vi "CSM-Logger-Thread.vi"(4 "Log Limit":T1={"file size (in bytes)"=10000000, "file num"=2} {"file size (in bytes)" format="%.0p"}, 6 "Exit When All Module Exist? (F)":bool, 7 "Format String":string="%<%Y/%m/%d %H:%M:%S%3u>T", 8 "error in (no error)":errorcluster, 9 "WatchDogQ":refnum<queue>, 10 "GlobalLogFilter.lvclass":refnum<class "LogFilter.lvclass">, 11 "File Path (Use Dialog)":path) -> (0 "error out":errorcluster)   [LabVIEW 2017, in "CSM File Logger.lvlib"]
doc: "The thread VI used in the CSM - Start File Logger VI.\n\n\n> [!NOTE] <b>CSM File Logger Implementation Principle</b>\n>\n> The CSM File Logger retrieves all execution records in the application via the CSM Global Log API and saves them to a specified text file for later analysis and error localization. The file format is a text file with the suffix `.csmlog`, which can be opened using text editing query tools such as Notepad."
uses:
  CSM File Logger.lvlib
  CSM File Logger Limit.ctl
  _Support/GlobalEvent/LogFilter/LogFilter.lvclass
  _Support/Typedef/_CSM_List Module Scope.ctl
  Communicable State Machine.lvlib
  _Shared/CSM Shared.lvlib
panel:
  in  "internal Stop":bool
  out "#MsgInQueue":i32
  out "size (in bytes)":i64
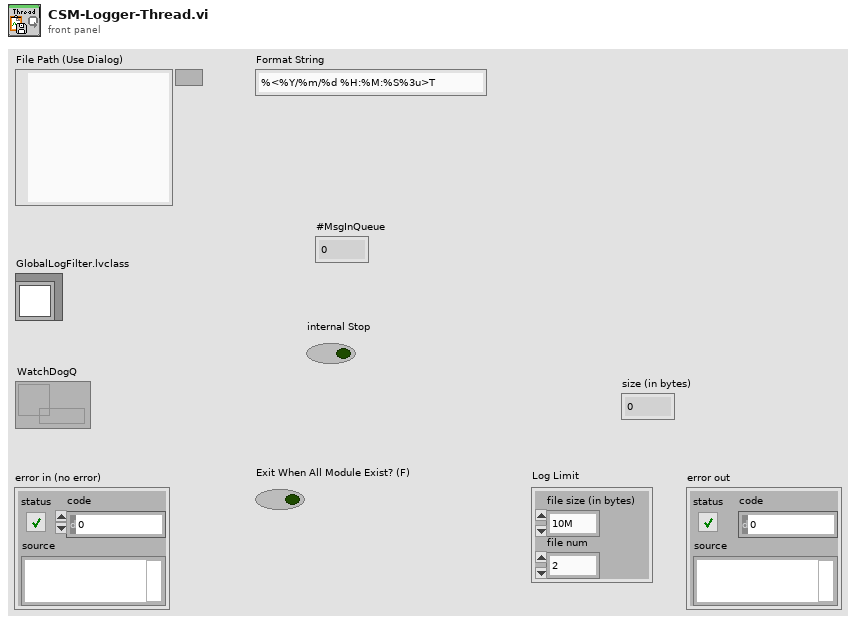
[diagram p1: front panel]
types:
  T1 = typedef "CSM File Logger.lvlib/CSM File Logger Limit.ctl" = cluster{"file size (in bytes)":i64, "file num":i32}
  T2 = typedef "Communicable State Machine.lvlib/_CSM_GlobalLog_MSG_TYPE.ctl" = enum16{"User Log", "State Change", "Status", "Interrupt", "Register", "Unregister", "Error Log", "Module Created", "Module Destroyed", "Async Message", "No-Rep Async Message", "Sync Message"}
  T3 = typedef "Communicable State Machine.lvlib/_CSM_GlobalLog_STATE_TYPE.ctl" = enum16{"State - Internal State", "State - External Message", "State - Response", "State - Complete"}
  T4 = cluster{"Global":cluster{"CSM":string[], "LogType":T2[], "State":string[], "StateType":T3[]}, "CSM":cluster{"LogType":cluster{"CSM":string, "LogType":T2}[], "State":cluster{"CSM":string, "State":string}[], "StateType":cluster{"CSM":string, "LogType":T3}[]}, "PeriodicLog":cluster{"Enable":bool, "Threshold(#/s)":dbl, "CheckPeriod(s)":dbl}}
  T5 = cluster{"Queue":path[], "folder":path, "name":string, "index":i32, "Log Limit":T1}
  T6 = enum16{"open", "replace", "create", "open or create", "replace or create", "replace or create with confirmation"}
  T7 = typedef "Communicable State Machine.lvlib/_CSM_List Module Scope.ctl" = enum16{"Normal", "System Only", "All"}
  T8 = typedef "Communicable State Machine.lvlib/Periodic String Filter Level.ctl" = enum16{"normal", "L1", "L2", "L3", "L4"}
  T9 = typedef "Communicable State Machine.lvlib/_CSM_GlobalLog_MSG.ctl" = cluster{"Name (\"\" to Use UUID)":string, "Current State":string, "Arguments":string, "Source Message":T10, "Source Module":string, "Complete(T)/Start(F)":bool, "LogType":T2, "Time Stamp":timestamp}
  T10 = typedef "Communicable State Machine.lvlib/_CSM_Response Source Message.ctl" = cluster{"‘State":string, "’Arguments":string, "’Error":errorcluster}
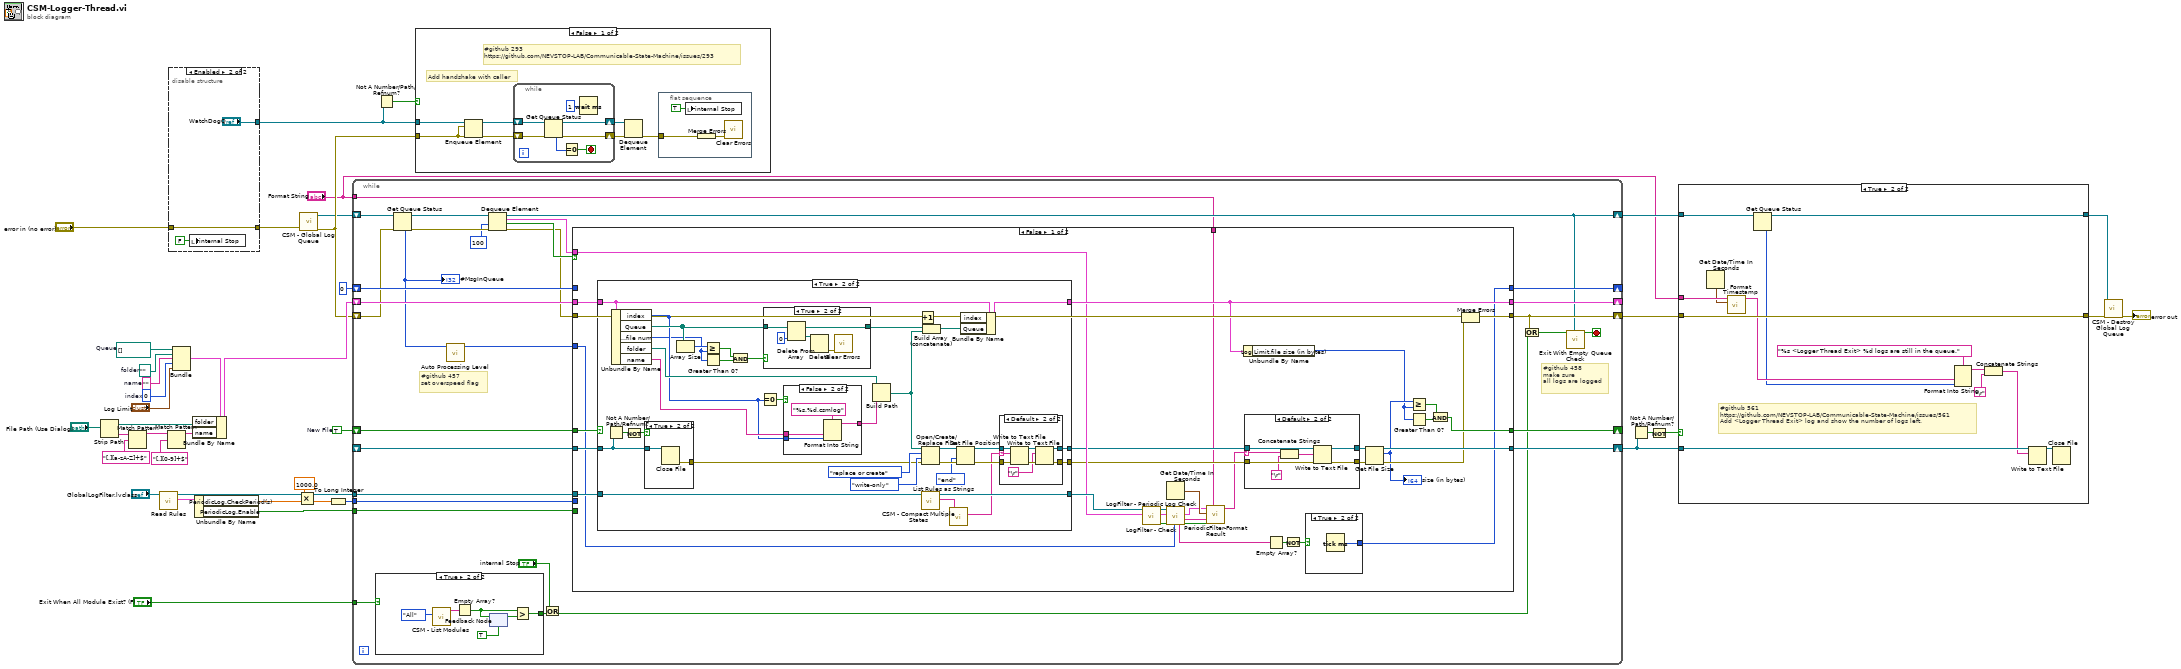
[diagram p0: block diagram]
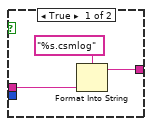
[diagram p6: hidden frame]
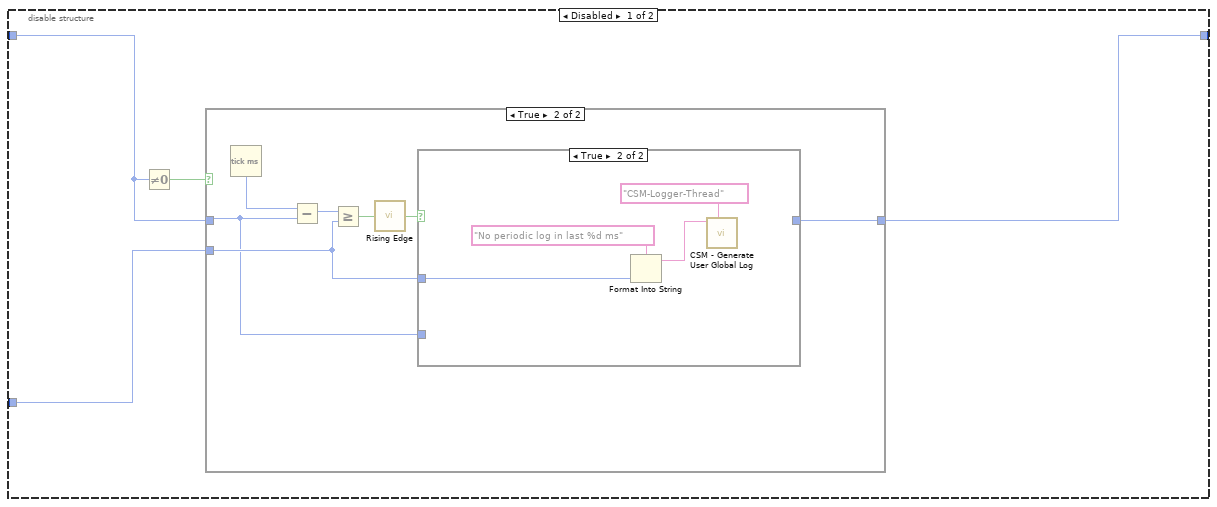
[diagram p10: hidden frame]
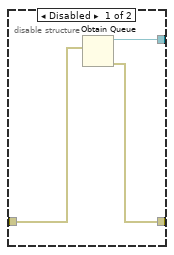
[diagram p15: hidden frame]
diagram:
  w28 = ""  # name
  w31 = 0  # index
  w32 = path ""  # folder
  w33 = path[] []  # Queue
  w34 = TRUE  # New File
  n1 = Strip Path(path="File Path (Use Dialog)") -> (stripped path=w21:path, name=w27:string)
  n2 = Match Pattern(string=w27, regular expression="[.][a-zA-Z]+$") -> (before substring=w24:string)  [unwired: 1 in, 3 out]
  n3 = call "Read Rules.vi"("LogFilter In"="GlobalLogFilter.lvclass") -> ("Rules"=w16:T4, "LogFilter Out"=w17:refnum<class "LogFilter.lvclass">)  [unwired: 8 in, 1 out]
  n4 = Match Pattern(string=w24, regular expression="[.][0-9]+$") -> (before substring=w22:string)  [unwired: 1 in, 3 out]
  n5 = disable-structure shown="Enabled" {
    disable-tunnel: [w41 "WatchDogQ"] -> w40
    disable-tunnel: [w43 w45] -> w6
    disable-tunnel: "error in (no error)" -> [w42 w45]
    frame Disabled {
      n6 = Obtain Queue(element data type=w42) -> (queue out=w41:refnum<queue>, error out=w43:errorcluster)  [unwired: 4 in, 1 out]
    }
    frame Enabled {
      n7 = local write "internal Stop"(FALSE ("internal Stop")) -> ()
    }
  }
  n8 = Bundle("Queue"=w33, "folder"=w32, "name"=w28, "index"=w31, "Log Limit"="Log Limit") -> (w29:T5)  [unwired: 1 in]
  n9 = Bundle By Name(cluster=w29, "folder"=w21, "name"=w22) -> (w23:T5)
  n10 = Unbundle By Name(w16) -> ("PeriodicLog.CheckPeriod(s)"=w14:dbl, "PeriodicLog.Enable"=w15:bool)
  n11 = Multiply(x=1000.0, y=w14) -> (x*y=w13:dbl)
  n12 = call "CSM - Global Log Queue.vi"("Error In"=w6) -> ("error out"=w9:errorcluster, "Global Log Queue"=w7:refnum<queue>)  [unwired: 9 in]
  n13 = To Long Integer(number=w13) -> (32bit integer=w11:i32)
  n14 = while {
    shift-right: [w76] -> w4
    shift-left: w9 -> [w59]
    shift-right: [w74] -> w36
    shift-left: _ -> [w75]
    tunnel: "Exit When All Module Exist? (F)" -> [w58]
    shift-right: [w72] -> _
    shift-left: w34 -> [w73]
    shift-right: [w70] -> _
    shift-left: w23 -> [w71]
    tunnel: w17 -> [w69]
    tunnel: w15 -> [w66]
    tunnel: w11 -> [w68]
    shift-right: [w67] -> _
    shift-left: u32 0 ("millisecond timer value") -> [w65]
    shift-right: [w50] -> w2
    shift-left: w7 -> [w62]
    tunnel: "Format String" -> [w47]
    stop <- w51 stop-if-true
    # "#github 458\nmake sure \nall logs are logged"
    # "#github 457\nset overspeed flag"
    n15 = case shown="True" w58 {
      tunnel: [_ w208] -> w57
      frame False {
      }
      frame True {
        n16 = call "CSM - List Modules.vi"("Scope (Normal)"=_CSM_List_Module_Scope."All" ("Mode")) -> ("Module Names"=w212:string[])  [unwired: 9 in, 1 out]
        n17 = Empty Array?(array=w212) -> (empty?=w211:bool)
        n18 = feedback #1(TRUE ("All?")) -> (w210:bool)
        n19 = feedback-in #1(w211) -> ()
        n20 = Greater?(x=w211, y=w210) -> (0:w208:bool)
      }
    }
    n21 = Get Queue Status(queue=w62, error in (no error)=w59) -> (queue out=w61:refnum<queue>, error out=w60:errorcluster, # elements in queue=w49:i32)  [unwired: 1 in, 5 out]
    "#MsgInQueue" <- w49
    n22 = call "Auto Processing Level.vi"("#Left In Q"=w49) -> ("Level"=w48:T8)  [unwired: 8 in, 2 out]
    n23 = Dequeue Element(queue=w61, timeout in ms (-1)=100, error in (no error)=w60) -> (queue out=w50:refnum<queue>, element=w53:T9, timed out?=w64:bool, error out=w63:errorcluster)
    n24 = Or(x="internal Stop", y=w57) -> (x .or. y?=w55:bool)
    n25 = case shown="False" w64 {
      tunnel: w63 -> [w110 w189]
      tunnel: [w109 w189] -> w76
      tunnel: w75 -> [w108 w188]
      tunnel: [w107 w188] -> w74
      tunnel: w73 -> [w106 w187]
      tunnel: [w105 w187] -> w72
      tunnel: w71 -> [w104 w186]
      tunnel: [w103 w186] -> w70
      tunnel: w69 -> [w102 _]
      tunnel: w68 -> [_ w185]
      tunnel: [w101 w183] -> w67
      tunnel: w66 -> [_ _]
      tunnel: w65 -> [_ w184]
      tunnel: w53 -> [w91 _]
      tunnel: w48 -> [w86 _]
      tunnel: w47 -> [w77 _]
      frame False {
        n26 = case shown="True" w106 {
          tunnel: w108 -> [w123 w155]
          tunnel: [_ w127] -> w88
          tunnel: [w123 w128] -> w87
          tunnel: [w122 w144] -> w103
          tunnel: w104 -> [w122 w146]
          tunnel: [w121 w126] -> w95
          tunnel: w102 -> [w121 w131]
          frame False {
          }
          frame True {
            n27 = Not A Number/Path/Refnum?(number/path/refnum=w155) -> (NaN/Path/Refnum?=w156:bool)
            n28 = Unbundle By Name(w146) -> ("index"=w136:i32, "Queue"=w147:path[], "Log Limit.file num"=w133:i32, "folder"=w140:path, "name"=w139:string)
            n29 = Not(x=w156) -> (.not. x?=w157:bool)
            n30 = case shown="True" w157 {
              tunnel: w155 -> [_ w182]
              tunnel: [_ w181] -> w149
              frame False {
              }
              frame True {
                n31 = Close File(refnum=w182) -> (error out=w181:errorcluster)  [unwired: 1 in, 1 out]
              }
            }
            n32 = Array Size(array=w147) -> (size(s)=w148:i32)
            n33 = Greater Or Equal?(x=w148, y=w133) -> (x >= y?=w135:bool)
            n34 = Greater Than 0?(x=w133) -> (x > 0?=w134:bool)
            n35 = And(x=w135, y=w134) -> (x .and. y?=w132:bool)
            n36 = Equal To 0?(x=w136) -> (x = 0?=w137:bool)
            n37 = case shown="True" w132 {
              tunnel: w147 -> [w175 w180]
              tunnel: [w175 w176] -> w145
              frame False {
              }
              frame True {
                n38 = Delete From Array(array=w180, index=0) -> (deleted portion=w178:path, array with subset deleted=w176:path[])  [unwired: 1 in]
                n39 = Delete(path (use dialog)=w178) -> (error out=w177:errorcluster)  [unwired: 4 in, 2 out]
                n40 = call <vilib>:"Clear Errors.vi"("error in (no error)"=w177) -> ()  [unwired: 5 in, 2 out]
              }
            }
            n41 = case shown="False" w137 {
              tunnel: [w169 w173] -> w141
              tunnel: w139 -> [w168 w172]
              tunnel: w136 -> [_ w171]
              frame True {
                n42 = Format Into String(format string="%s.csmlog", w168) -> (resulting string=w169:string)  [unwired: 2 in, 1 out]
              }
              frame False {
                n43 = Format Into String(format string="%s.%d.csmlog", w172, w171) -> (resulting string=w173:string)  [unwired: 2 in, 1 out]
              }
            }
            n44 = Build Path(base path=w140, name or relative path=w141) -> (appended path=w138:path)
            n45 = Increment(x=w136) -> (x+1=w142:i32)
            n46 = call "List Rules as Strings.vi"("GlobalLogFilter In"=w131) -> ("Rule Strings"=w125:string[], "GlobalLogFilter Out"=w126:refnum<class "LogFilter.lvclass">)  [unwired: 8 in, 1 out]
            n47 = Open/Create/Replace File(file path (use dialog)=w138, error in=w149, operation (0:open)=T6."replace or create", access (0:read/write)=enum16{"read/write", "read-only", "write-only"}."write-only") -> (refnum out=w154:refnum<file>, error out=w153:errorcluster)  [unwired: 2 in, 1 out]
            n48 = Build Array (concatenate)(w145, w138) -> (w143:path[])
            n49 = call "CSM - Compact Multiple States.vi"("Multiple States"=w125) -> ("States"=w124:string)  [unwired: 9 in]
            n50 = Set File Position(refnum=w154, from (0:start)=enum16{"start", "end", "current"}."end", error in=w153) -> (refnum out=w129:refnum<file>, error out=w130:errorcluster)  [unwired: 1 in]
            n51 = Bundle By Name(cluster=w146, "index"=w142, "Queue"=w143) -> (w144:T5)
            n52 = case shown="Default" w124 {
              selector: w124 -> [_ w167]
              tunnel: w130 -> [w158 w166]
              tunnel: w129 -> [w159 w165]
              tunnel: [w159 w162] -> w128
              tunnel: [w158 w161] -> w127
              frame "" {
              }
              frame Default {
                n53 = Write to Text File(file (use dialog)=w165, text=w167, error in=w166) -> (refnum out=w163:refnum<file>, error out=w164:errorcluster)  [unwired: 1 in, 1 out]
                n54 = Write to Text File(file (use dialog)=w163, text="\r", error in=w164) -> (refnum out=w162:refnum<file>, error out=w161:errorcluster)  [unwired: 1 in, 1 out]
              }
            }
          }
        }
        n55 = call "LogFilter - Check.vi"("Cross CSM Data In"=w91, "GlobalLogFilter In"=w95) -> ("Matched? (Dup)"=w82:bool, "Cross CSM Data Out"=w83:T9, "GlobalLogFilter.lvclass (Dup)"=w84:refnum<class "LogFilter.lvclass">)  [unwired: 7 in]
        n56 = Get Date/Time In Seconds() -> (seconds since 1Jan1904=w85:timestamp)
        n57 = call "LogFilter - Periodic Log Check.vi"("Level (Normal)"=w86, "Matched Previous?"=w82, "Cross CSM Data In"=w83, "GlobalLogFilter In"=w84) -> ("Matched? (Dup)"=w79:bool, "Additional Info"=w80:string[], "Cross CSM Data Out"=w81:T9, "Filtered Status"=w94:string[])  [unwired: 3 in, 1 out]
        n58 = call "PeriodicFilter-Format Result.vi"("Time Format String"=w77, "Filtered"=w79, "Additional Info"=w80, "Current Time"=w85, "Cross CSM Data In"=w81) -> ("States"=w78:string)  [unwired: 6 in]
        n59 = Unbundle By Name(w103) -> ("Log Limit.file size (in bytes)"=w96:i64)
        n60 = case shown="Default" w78 {
          selector: w78 -> [_ w114]
          tunnel: w88 -> [w111 w119]
          tunnel: w87 -> [w112 w118]
          tunnel: [w112 w117] -> w90
          tunnel: [w111 w116] -> w89
          frame "" {
          }
          frame Default {
            n61 = Concatenate Strings(w114, "\r") -> (w113:string)
            n62 = Write to Text File(file (use dialog)=w118, text=w113, error in=w119) -> (refnum out=w117:refnum<file>, error out=w116:errorcluster)  [unwired: 1 in, 1 out]
          }
        }
        n63 = Empty Array?(array=w94) -> (empty?=w93:bool)
        n64 = Not(x=w93) -> (.not. x?=w92:bool)
        n65 = case shown="True" w92 {
          tunnel: [_ w120] -> w101
          frame False {
          }
          frame True {
            n66 = Tick Count (ms)() -> (millisecond timer value=w120:u32)
          }
        }
        n67 = Get File Size(file=w90, error in=w89) -> (refnum out=w107:refnum<file>, size (in bytes)=w99:i64, 0:w100:errorcluster)
        "size (in bytes)" <- w99
        n68 = Greater Or Equal?(x=w99, y=w96) -> (x >= y?=w98:bool)
        n69 = Greater Than 0?(x=w96) -> (x > 0?=w97:bool)
        n70 = And(x=w98, y=w97) -> (x .and. y?=w105:bool)
        n71 = Merge Errors(w110, w100) -> (w109:errorcluster)
      }
      frame True {
        n72 = disable-structure shown="Enabled" {
          disable-tunnel: w185 -> [w193 _]
          disable-tunnel: w184 -> [w192 _]
          disable-tunnel: [w190 _] -> w183
          frame Disabled {
            n73 = Not Equal To 0?(x=w192) -> (x != 0?=w191:bool)
            n74 = case shown="True" w191 {
              tunnel: w192 -> [w194 w197]
              tunnel: w193 -> [_ w199]
              tunnel: [w194 w198] -> w190
              frame False {
              }
              frame True {
                n75 = Tick Count (ms)() -> (millisecond timer value=w201:u32)
                n76 = Subtract(x=w201, y=w197) -> (x-y=w200:u32)
                n77 = Greater Or Equal?(x=w200, y=w199) -> (x >= y?=w196:bool)
                n78 = call "Rising Edge.vi"("Signal"=w196) -> ("Rising Edge"=w195:bool)
                n79 = case shown="True" w195 {
                  tunnel: w199 -> [_ w203]
                  tunnel: [w202 _] -> w198
                  tunnel: w197 -> [w202 _]
                  frame False {
                  }
                  frame True {
                    n80 = Format Into String(format string="No periodic log in last %d ms" ("Log"), w203) -> (resulting string=w204:string)  [unwired: 2 in, 1 out]
                    n81 = call "CSM - Generate User Global Log.vi"("Place (\"\" to Use VI's Name)"="CSM-Logger-Thread" ("Place(\"\" to use VI's Name)"), "Log"=w204) -> ()  [unwired: 9 in, 1 out]
                  }
                }
              }
            }
          }
          frame Enabled {
          }
        }
      }
    }
    n82 = Or(x=w76, y=w55) -> (x .or. y?=w52:bool)
    n83 = call "Exit With Empty Queue Check.vi"("Queue"=w50, "Stop"=w52) -> ("Exit"=w51:bool)  [unwired: 8 in, 1 out]
  }
  n84 = Not A Number/Path/Refnum?(number/path/refnum=w40) -> (NaN/Path/Refnum?=w39:bool)
  n85 = case shown="False" w39 {
    tunnel: w40 -> [w218 _]
    tunnel: w9 -> [w213 _]
    frame False {
      # "#github 293 \nhttps://github.com/NEVSTOP-LAB/Communicable-State-Machine/issues/293"
      # "Add handshake with caller"
      n86 = Enqueue Element(queue=w218, element=w213, error in (no error)=w213) -> (queue out=w217:refnum<queue>, error out=w215:errorcluster)  [unwired: 1 in, 1 out]
      n87 = while {
        shift-right: [w225] -> w216
        shift-left: w217 -> [w226]
        shift-right: [w223] -> w214
        shift-left: w215 -> [w224]
        stop <- w221 stop-if-true
        n88 = Get Queue Status(queue=w226, error in (no error)=w224) -> (queue out=w225:refnum<queue>, error out=w223:errorcluster, # elements in queue=w222:i32)  [unwired: 1 in, 5 out]
        n89 = Equal To 0?(x=w222) -> (x = 0?=w221:bool)
        n90 = Wait (ms)(milliseconds to wait=u32 1) -> ()  [unwired: 1 out]
      }
      n91 = Dequeue Element(queue=w216, error in (no error)=w214) -> (error out=w219:errorcluster)  [unwired: 1 in, 3 out]
      n92 = flat-sequence {
        tunnel: w219 -> [w229]
        frame #0 {
          n93 = local write "internal Stop"(TRUE ("internal Stop")) -> ()
          n94 = Merge Errors(w229) -> (w228:errorcluster)
          n95 = call <vilib>:"Clear Errors.vi"("error in (no error)"=w228) -> ()  [unwired: 5 in, 2 out]
        }
      }
    }
    frame True {
    }
  }
  n96 = Not A Number/Path/Refnum?(number/path/refnum=w36) -> (NaN/Path/Refnum?=w37:bool)
  n97 = Not(x=w37) -> (.not. x?=w35:bool)
  n98 = case shown="True" w35 {
    tunnel: w36 -> [_ w244]
    tunnel: [w230 w242] -> w5
    tunnel: w4 -> [w230 w242]
    tunnel: [w231 w234] -> w3
    tunnel: w2 -> [w231 w241]
    tunnel: "Format String" -> [_ w238]
    frame False {
    }
    frame True {
      # "#github 561\nhttps://github.com/NEVSTOP-LAB/Communicable-State-Machine/issues/561\nAdd <Logger Thread Exit> log and show the number of logs left."
      n99 = Get Date/Time In Seconds() -> (seconds since 1Jan1904=w237:timestamp)
      n100 = call "Format Timestamp.vi"("Timestamp"=w237, "Format String"=w238) -> ("String"=w233:string)  [unwired: 9 in]
      n101 = Get Queue Status(queue=w241) -> (queue out=w234:refnum<queue>, # elements in queue=w232:i32)  [unwired: 2 in, 6 out]
      n102 = Format Into String(format string="%s <Logger Thread Exit> %d logs are still in the queue.", w233, w232) -> (resulting string=w235:string)  [unwired: 2 in, 1 out]
      n103 = Concatenate Strings(w235, "\r") -> (w239:string)
      n104 = Write to Text File(file (use dialog)=w244, text=w239) -> (refnum out=w243:refnum<file>)  [unwired: 2 in, 2 out]
      n105 = Close File(refnum=w243) -> ()  [unwired: 1 in, 2 out]
    }
  }
  n106 = call "CSM - Destroy Global Log Queue.vi"("Error In"=w5, "Global Log Queue"=w3) -> ("error out"=→"error out":errorcluster)  [unwired: 9 in]
